vi "RichToFlatlv_python_grpc_webui_demo_v1_HeaterStateUpdated.vi"(5 "OutputClusterType":T1, 11 "InputCluster":T3) -> (3 "OutputCluster":T1)   [LabVIEW 2020, in "thermal-chamber-controller_server.lvlib"]
uses:
  thermal-chamber-controller_server.lvlib
  lv_python_grpc_webui_demo_v1_HeaterStateUpdated.ctl
  lv_python_grpc_webui_demo_v1_HeaterState.ctl
  lv_python_grpc_webui_demo_v1_HeaterStateUpdated_Flat.ctl
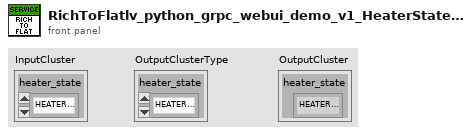
[diagram p1: front panel]
types:
  T1 = typedef "thermal-chamber-controller_server.lvlib/lv_python_grpc_webui_demo_v1_HeaterStateUpdated_Flat.ctl" = cluster{"heater_state":T2}
  T2 = typedef "thermal-chamber-controller_server.lvlib/lv_python_grpc_webui_demo_v1_HeaterState.ctl" = enum32{"HEATER_ENABLED", "HEATER_DISABLED"}
  T3 = typedef "thermal-chamber-controller_server.lvlib/lv_python_grpc_webui_demo_v1_HeaterStateUpdated.ctl" = cluster{"heater_state":T2}
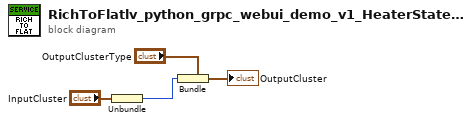
[diagram p0: block diagram]
diagram:
  n1 = Unbundle "Unbundle"("InputCluster") -> ("heater_state"=w1:T2)
  n2 = Bundle "Bundle"(cluster="OutputClusterType", "heater_state"=w1) -> (→"OutputCluster":T1)
